vi "post-suite action.vi"(8 "error in (no error)":errorcluster, 11 "Test Runner.JUnit in":refnum<class "Test Runner.JUnit.lvclass">) -> (0 "error out":errorcluster, 3 "Test Runner.JUnit out":refnum<class "Test Runner.JUnit.lvclass">)   [LabVIEW 2020, in "Test Runner.JUnit.lvclass"]
uses:
  Test Runner.JUnit.lvclass
  Test Runner.JUnit.lvclass/Test Runner.JUnit.ctl
  classes/Test Runner/Test Runner.lvclass
  <vilib>/regexp/Match Regular Expression.xnode
  classes/Test/Test.lvclass
  classes/Assert/Assert.lvclass
panel:
  out "substring 2":string
  out "substring":string
  out "text":string
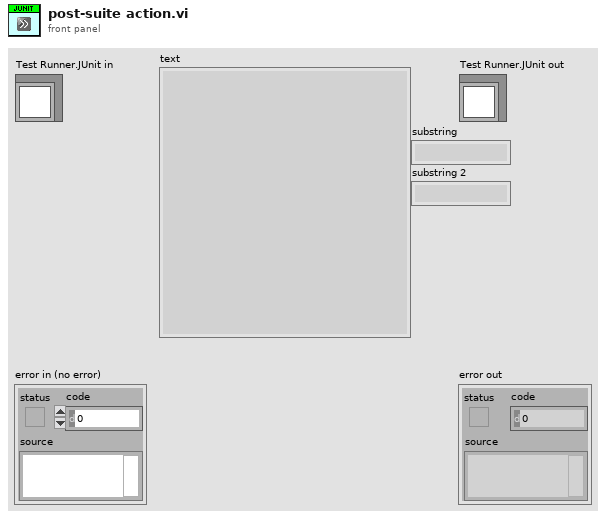
[diagram p1: front panel]
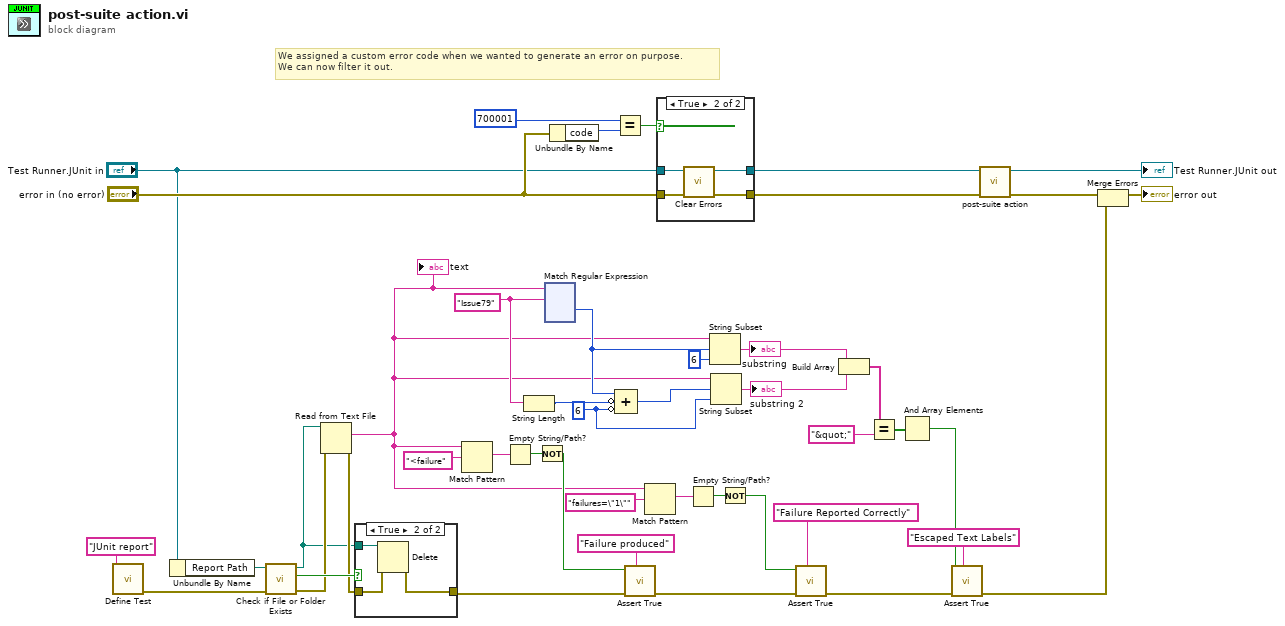
[diagram p0: block diagram]
diagram:
  w16 = 6 ("length (rest)")
  w28 = "Issue79" ("regular expression")
  # "We assigned a custom error code when we wanted to generate an error on purpose.\nWe can now filter it out."
  n1 = call "Define Test.vi"("Label (VI Title)"="JUnit report") -> ("error out"=w36:errorcluster)  [unwired: 9 in, 1 out]
  n2 = Unbundle By Name("Test Runner.JUnit in") -> ("Report Path"=w37:path)
  n3 = call <vilib>:"Check if File or Folder Exists.vi"("error in (no error)"=w36, "path"=w37) -> ("error out"=w43:errorcluster, "file or folder exists?"=w44:bool, "dup path"=w41:path)  [unwired: 7 in]
  n4 = Read from Text File(file (use dialog)=w41, error in=w43) -> (text=w5:string, error out=w42:errorcluster)  [unwired: 2 in, 2 out]
  "text" <- w5
  n5 = case shown="True" w44 {
    tunnel: w41 -> [_ w49]
    tunnel: w42 -> [w46 w48]
    tunnel: [w46 w47] -> w33
    frame False {
    }
    frame True {
      n6 = Delete(path (use dialog)=w49, error in=w48) -> (error out=w47:errorcluster)  [unwired: 3 in, 2 out]
    }
  }
  n7 = Match Pattern(string=w5, regular expression="<failure") -> (match substring=w39:string)  [unwired: 1 in, 3 out]
  n8 = Empty String/Path?(string/path=w39) -> (empty?=w38:bool)
  n9 = String Length(string=w28) -> (length=w26:i32)
  n10 = Not(x=w38) -> (.not. x?=w34:bool)
  n11 = xnode ("Match Regular Expression")("input string"=w5, "regular expression"=w28) -> ("offset past match"=w27:i32)  [unwired: 4 in, 4 out]
  n12 = Unbundle By Name("error in (no error)") -> ("code"=w15:i32)
  n13 = Equal?(x=700001 ("error code (1)"), y=w15) -> (x = y?=w13:bool)
  n14 = Compound Arithmetic op=ADD(w27, invert w26, invert w16) -> (w25:i32)
  n15 = call "Assert True.vi"("Label"="Failure produced", "error in (no error)"=w33, "True?"=w34) -> ("error out"=w4:errorcluster)  [unwired: 7 in, 1 out]
  n16 = Match Pattern(string=w5, regular expression="failures=\"1\"") -> (match substring=w7:string)  [unwired: 1 in, 3 out]
  n17 = case shown="True" w13 {
    tunnel: "error in (no error)" -> [w50 w54]
    tunnel: [w50 w53] -> w11
    tunnel: [w51 w52] -> w10
    tunnel: "Test Runner.JUnit in" -> [w51 w52]
    frame False {
    }
    frame True {
      n18 = call <vilib>:"Clear Errors.vi"("error in (no error)"=w54) -> ("error out"=w53:errorcluster)  [unwired: 5 in, 1 out]
    }
  }
  n19 = Empty String/Path?(string/path=w7) -> (empty?=w8:bool)
  n20 = String Subset(string=w5, offset (0)=w27, length (rest)=6 ("length (rest)")) -> (substring=w24:string)
  "substring" <- w24
  n21 = String Subset(string=w5, offset (0)=w25, length (rest)=w16) -> (substring=w23:string)
  "substring 2" <- w23
  n22 = Not(x=w8) -> (.not. x?=w2:bool)
  n23 = call "Assert True.vi"("Label"="Failure Reported Correctly", "error in (no error)"=w4, "True?"=w2) -> ("error out"=w3:errorcluster)  [unwired: 7 in, 1 out]
  n24 = Build Array(w24, w23) -> (w21:string[])
  n25 = Equal?(x=w21, y="&quot;" ("regular expression")) -> (x = y?=w19:bool[])
  n26 = And Array Elements(Boolean array=w19) -> (logical AND=w18:bool)
  n27 = call "Assert True.vi"("Label"="Escaped Text Labels", "error in (no error)"=w3, "True?"=w18) -> ("error out"=w22:errorcluster)  [unwired: 7 in, 1 out]
  n28 = call-parent "post-suite action.vi"("error in (no error)"=w11, "Test Runner in"=w10) -> ("error out"=w32:errorcluster, "Test Runner out"=→"Test Runner.JUnit out":refnum<class "Test Runner.JUnit.lvclass">)  [unwired: 8 in]
  n29 = Merge Errors(w32, w22) -> (→"error out":errorcluster)
